vi "csb max frames.vi"(8 "error in (no error)":errorcluster, 11 "in_len":i32) -> (0 "error out":errorcluster, 3 "function return":i32)   [LabVIEW 2021, in "CANsub_Codec.lvlib"]
doc: "int32_t csb_max_frames(int32_t in_len);"
uses:
  CANsub_Codec.lvlib
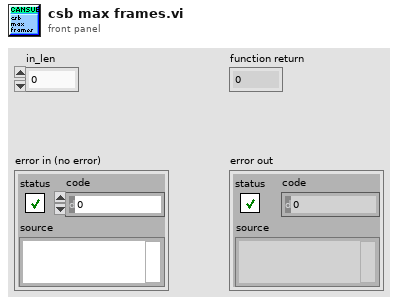
[diagram p1: front panel]
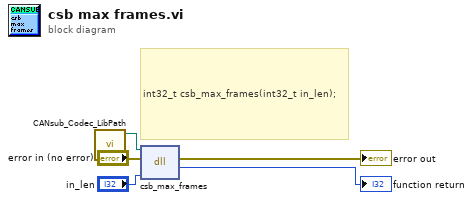
[diagram p0: block diagram]
diagram:
  # "int32_t csb_max_frames(int32_t in_len);"
  n1 = call "CANsub_Codec_LibPath.vi"() -> ("Path"=w1:path)  [unwired: 11 in]
  n2 = dll-call lib="libcansub_codec.*" fn="csb_max_frames"(path in=w1, error in="error in (no error)", "in_len"="in_len") -> (error out=→"error out":errorcluster, "return type"=→"function return":i32)  [unwired: 2 in, 1 out]
